vi "VIH Constant - ProductInfo Keywords.vi"() -> (2 "ProductInfo keywords":string[](array[string]), 3 "Keyword description":string[](array[string]))   [LabVIEW 2014]
doc: "::: VI Helpeks :::\nCopyright (c) 2000-2026 Konstantin Shifershteyn. All rights reserved."
panel:
  # "VI Helpeks\nCopyright (c) 2012-2026 Konstantin Shifershteyn"
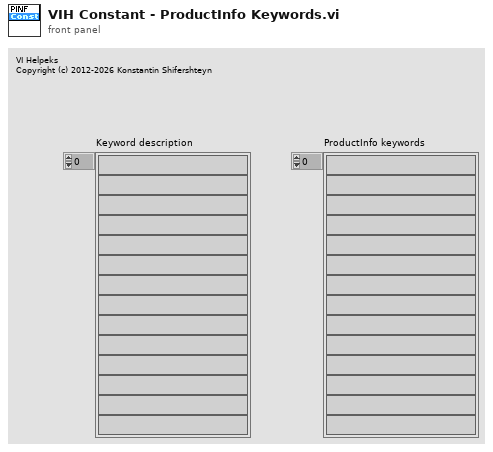
[diagram p1: front panel]
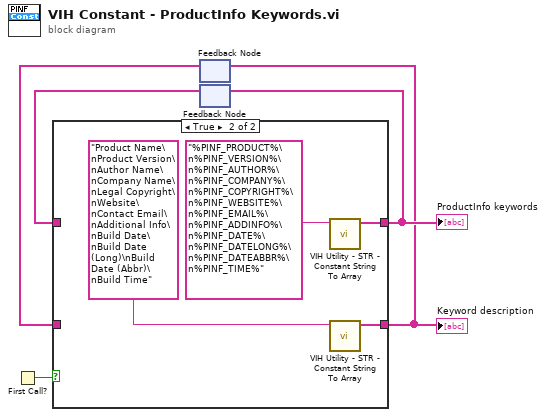
[diagram p0: block diagram]
diagram:
  n1 = First Call?() -> (First Call?: T/F=w5:bool)
  n2 = feedback #1() -> (w1:string[])  [unwired: 1 in]
  n3 = feedback #2() -> (w3:string[])  [unwired: 1 in]
  n4 = case shown="True" w5 {
    tunnel: [w7 w10] -> w4
    tunnel: [w6 w9] -> w2
    tunnel: w3 -> [w7 _]
    tunnel: w1 -> [w6 _]
    frame False {
    }
    frame True {
      n5 = call "VIH Utility - STR - Constant String To Array.vi"("String in"="%PINF_PRODUCT%\n%PINF_VERSION%\n%PINF_AUTHOR%\n%PINF_COMPANY%\n%PINF_COPYRIGHT%\n%PINF_WEBSITE%\n%PINF_EMAIL%\n%PINF_ADDINFO%\n%PINF_DATE%\n%PINF_DATELONG%\n%PINF_DATEABBR%\n%PINF_TIME%") -> ("Array out"=w10:string[])  [unwired: 10 in]
      n6 = call "VIH Utility - STR - Constant String To Array.vi"("String in"="Product Name\nProduct Version\nAuthor Name\nCompany Name\nLegal Copyright\nWebsite\nContact Email\nAdditional Info\nBuild Date\nBuild Date (Long)\nBuild Date (Abbr)\nBuild Time") -> ("Array out"=w9:string[])  [unwired: 10 in]
    }
  }
  "ProductInfo keywords" <- w4
  "Keyword description" <- w2
  n7 = feedback-in #1(w2) -> ()
  n8 = feedback-in #2(w4) -> ()
